vi "Own20261013_ReadClassFields.vi"() -> ()   [LabVIEW 2024]
uses:
  <resource>/Framework/Providers/MessageMakerProvider/_Message Maker/Message Maker.lvlib
panel:
  out "error out":errorcluster caption="错误输出"
  out "control_ids":refnum<vi>[](array[refnum])
  in  "Target Path":path
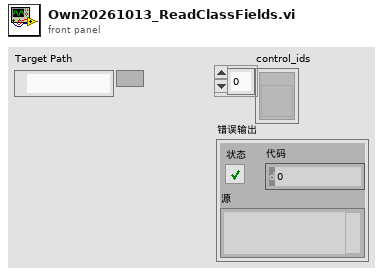
[diagram p1: front panel]
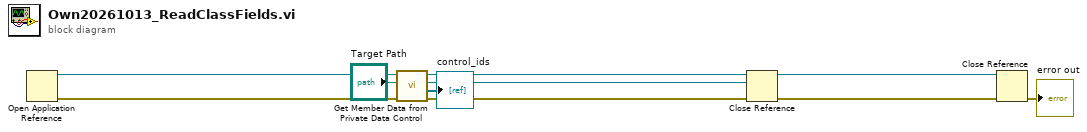
[diagram p0: block diagram]
diagram:
  n1 = Open Application Reference() -> (0:w5:errorcluster, 3:w6:refnum<vi>)  [unwired: 4 in]
  n2 = call <resource>:"Get Member Data from Private Data Control.vi"("AppInst"=w6, "error in (no error)"=w5, "Target Path"="Target Path") -> ("error out"=w3:errorcluster, "Controls"=→"control_ids":refnum<vi>[], "Private data Control"=w4:refnum<vi>)  [unwired: 6 in]
  n3 = Close Reference(reference=w4, error in (no error)=w3) -> (error out=w2:errorcluster)
  n4 = Close Reference(reference=w6, error in (no error)=w2) -> (error out=→"error out":errorcluster)
